vi "Get ECAT IOVs.vi"(8 "error in (no error)":errorcluster, 11 "ECAT Slave in":refnum<k21>="ni.var.io://localhost/EtherCAT Master/Device") -> (0 "error IO":errorcluster, 1 "All Mods":refnum<k21>[](array[refnum]), 2 "UDV Container":refnum<k21>[](array[refnum]), 3 "ECAT Slave out":refnum<k21>="ni.var.io:/", 5 "ECAT Variablenobjekt":refnum<k21>[](array[refnum]))   [LabVIEW 2027, in "SEECD Engine.lvlib"]
uses:
  SEECD Engine.lvlib
  <resource>/objmgr/IndComECAT.rc
  <resource>/objmgr/ni.var.rc
  <resource>/objmgr/cRIO.rc
  <vilib>/NI VeriStand/Custom Device Tools/Custom Device Utility Library/Custom Device Utility Library.lvlib
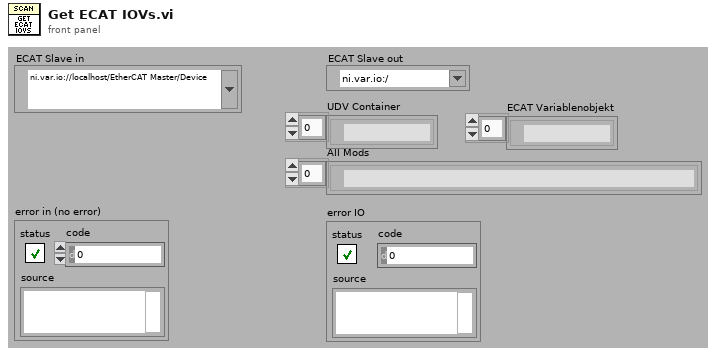
[diagram p1: front panel]
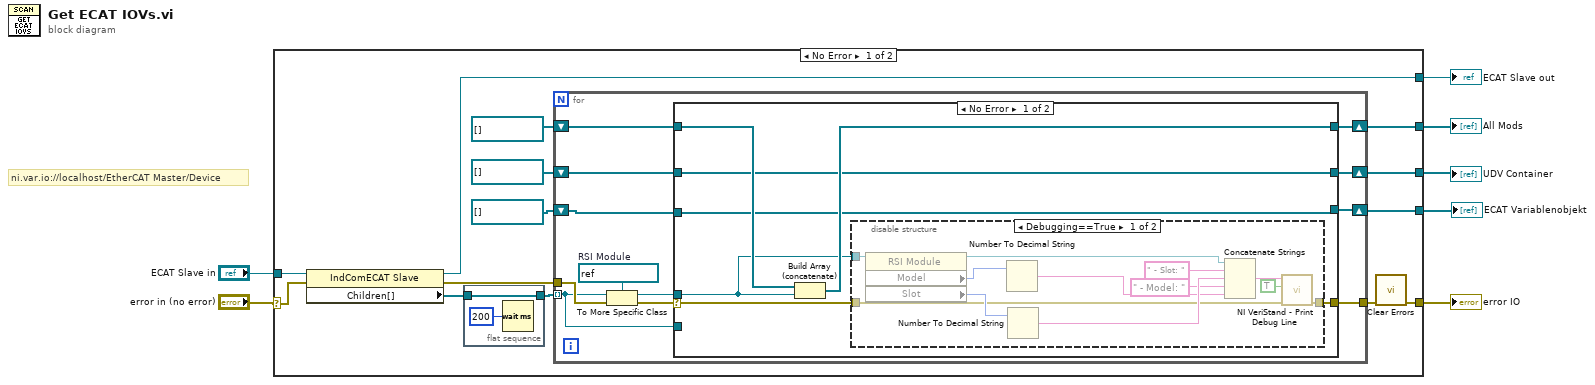
[diagram p0: block diagram]
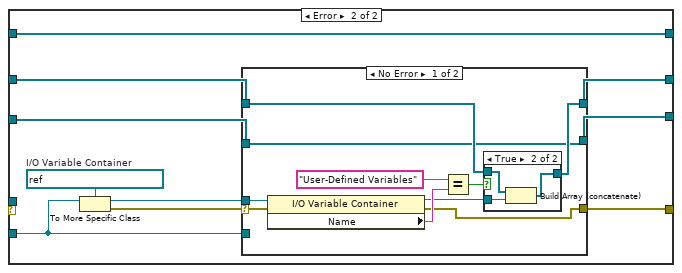
[diagram p3: hidden frame]
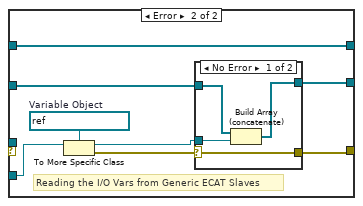
[diagram p5: hidden frame]
diagram:
  # "ni.var.io://localhost/EtherCAT Master/Device"
  n1 = case shown="No Error" "error in (no error)" {
    selector: "error in (no error)" -> [w18 w95]
    tunnel: [w21 w95] -> w7
    tunnel: [w15 _] -> w3
    tunnel: "ECAT Slave in" -> [w20 w94]
    tunnel: [w19 w94] -> w5
    tunnel: [w12 _] -> w2
    tunnel: [w8 _] -> w1
    frame No Error {
      n2 = property class="IndComECAT Slave"(reference=w20, error in=w18) -> (reference out=w19:refnum<k21>, error out=w16:errorcluster, "Children[]"=w11:refnum<k21>[])
      n3 = flat-sequence {
        tunnel: w11 -> [w23]
        tunnel: [w23] -> w10
        frame #0 {
          n4 = Wait (ms)(milliseconds to wait=u32 200) -> ()  [unwired: 1 out]
        }
      }
      n5 = for {
        tunnel: w10 -> [w26] mode=indexing
        tunnel: w16 -> [w35]
        shift-right: [w33] -> w15
        shift-left: refnum<k21>[] [] -> [w32]
        tunnel: [w31] -> w14
        shift-right: [w27] -> w12
        shift-left: refnum<k21>[] [] -> [w28]
        shift-right: [w25] -> w8
        shift-left: refnum<k21>[] [] -> [w24]
        w34 = refnum<k21> refnum  # RSI Module
        n6 = To More Specific Class(target class=w34, reference=w26, error in=w35) -> (specific class reference=w29:refnum<k21>, error out=w30:errorcluster)
        n7 = case shown="No Error" w30 {
          selector: w30 -> [w38 _]
          tunnel: w29 -> [w36 _]
          tunnel: [w42 w65] -> w33
          tunnel: w32 -> [w41 w65]
          tunnel: [w39 w59] -> w31
          tunnel: w28 -> [w40 w61]
          tunnel: [w40 w60] -> w27
          tunnel: w26 -> [_ w58]
          tunnel: [w37 w57] -> w25
          tunnel: w24 -> [w37 w56]
          frame No Error {
            n8 = Build Array (concatenate)(w41, w36) -> (w42:refnum<k21>[])
            n9 = disable-structure shown="Debugging==True" {
              disable-tunnel: [w48 w55] -> w39
              disable-tunnel: w38 -> [w47 w55]
              disable-tunnel: w36 -> [w44 _]
              frame condition #0 {
                n10 = property class="RSI Module"(reference=w44) -> (reference out=w45:refnum<k21>, "Model"=w54:u32, "Slot"=w53:u32)  [unwired: 1 in, 1 out]
                n11 = Number To Decimal String(number=w54) -> (decimal integer string=w49:string)  [unwired: 1 in]
                n12 = Number To Decimal String(number=w53) -> (decimal integer string=w51:string)  [unwired: 1 in]
                n13 = Concatenate Strings(w45, " - Slot: " ("string"), w51, " - Model: " ("string"), w49) -> (w46:string)
                n14 = call <vilib>:"NI VeriStand - Print Debug Line.vi"("error in (no error)"=w47, "Add to log file? (F)"=TRUE, "Message"=w46) -> ("error out"=w48:errorcluster)  [unwired: 8 in]
              }
              frame condition #1 (active) {
              }
            }
          }
          frame Error {
            w64 = refnum<k21> refnum  # I/O Variable Container
            n15 = To More Specific Class(target class=w64, reference=w58) -> (specific class reference=w62:refnum<k21>, error out=w63:errorcluster)  [unwired: 1 in]
            n16 = case shown="No Error" w63 {
              selector: w63 -> [w75 _]
              tunnel: [w69 w87] -> w60
              tunnel: w62 -> [w74 _]
              tunnel: [w68 w83] -> w59
              tunnel: w61 -> [w67 w87]
              tunnel: w58 -> [_ w82]
              tunnel: [w66 w81] -> w57
              tunnel: w56 -> [w66 w80]
              frame No Error {
                n17 = property class="I/O Variable Container"(reference=w74, error in=w75) -> (reference out=w70:refnum<k21>, error out=w68:errorcluster, "Name"=w73:string)
                n18 = Equal?(x="User-Defined Variables", y=w73) -> (x = y?=w71:bool)
                n19 = case shown="True" w71 {
                  tunnel: w70 -> [_ w78]
                  tunnel: w67 -> [w76 w79]
                  tunnel: [w76 w77] -> w69
                  frame False {
                  }
                  frame True {
                    n20 = Build Array (concatenate)(w79, w78) -> (w77:refnum<k21>[])
                  }
                }
              }
              frame Error {
                w84 = refnum<k21> refnum  # Variable Object
                # "Reading the I/O Vars from Generic ECAT Slaves"
                n21 = To More Specific Class(target class=w84, reference=w82) -> (specific class reference=w86:refnum<k21>, error out=w85:errorcluster)  [unwired: 1 in]
                n22 = case shown="No Error" w85 {
                  selector: w85 -> [w88 w93]
                  tunnel: [w91 w92] -> w81
                  tunnel: w86 -> [w90 _]
                  tunnel: w80 -> [w89 w92]
                  tunnel: [w88 w93] -> w83
                  frame No Error {
                    n23 = Build Array (concatenate)(w89, w90) -> (w91:refnum<k21>[])
                  }
                  frame Error {
                  }
                }
              }
            }
          }
        }
      }
      n24 = call <vilib>:"Clear Errors.vi"("error in (no error)"=w14) -> ("error out"=w21:errorcluster)  [unwired: 5 in, 1 out]
    }
    frame Error {
    }
  }
  "error IO" <- w7
  "ECAT Slave out" <- w5
  "All Mods" <- w3
  "UDV Container" <- w2
  "ECAT Variablenobjekt" <- w1
